vi "OwnMergeDiagram_75a8ff880a4e45db8adbb9b45fd37ec5.vi"() -> ()   [LabVIEW 2024]
doc: "该范例演示VI脚本的“移动选定对象”方法，以编程方式在编辑环境下触发鼠标拖动。这是移动多个对象的有效方法。\n\n将'Duplicate?'参数的值设置为TRUE，移动操作就可以成为复制操作。"
uses:
  <vilib>/Utility/miscctls.llb/LVDeltaXY32Cluster.ctl
panel:
  out "selected_source_objects":refnum<vi>[](array[refnum])
  out "error out":errorcluster caption="错误输出"
  in  "delta":T1 caption="X/Y Delta"
  in  "target_path":path
  in  "source_path":path
  # "概述：演示VI脚本中的移动选定对象方法，将当前选定区域移动至其他位置\n操作步骤：\n1.打开Test - Selection List Target.vi的程序框图。\n2.选择一个或多个对象。\n3.运行本VI。选中的对象将在程序框图上向上移动25个像素。"
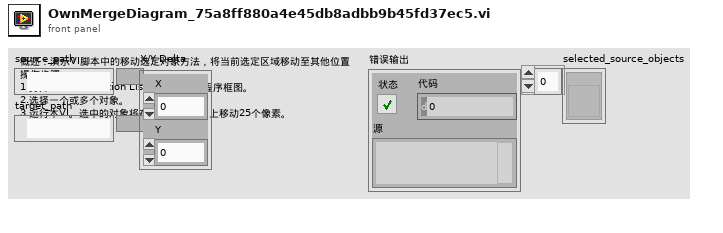
[diagram p1: front panel]
types:
  T1 = typedef "LVDeltaXY32Cluster.ctl" = cluster{"X":i32, "Y":i32}
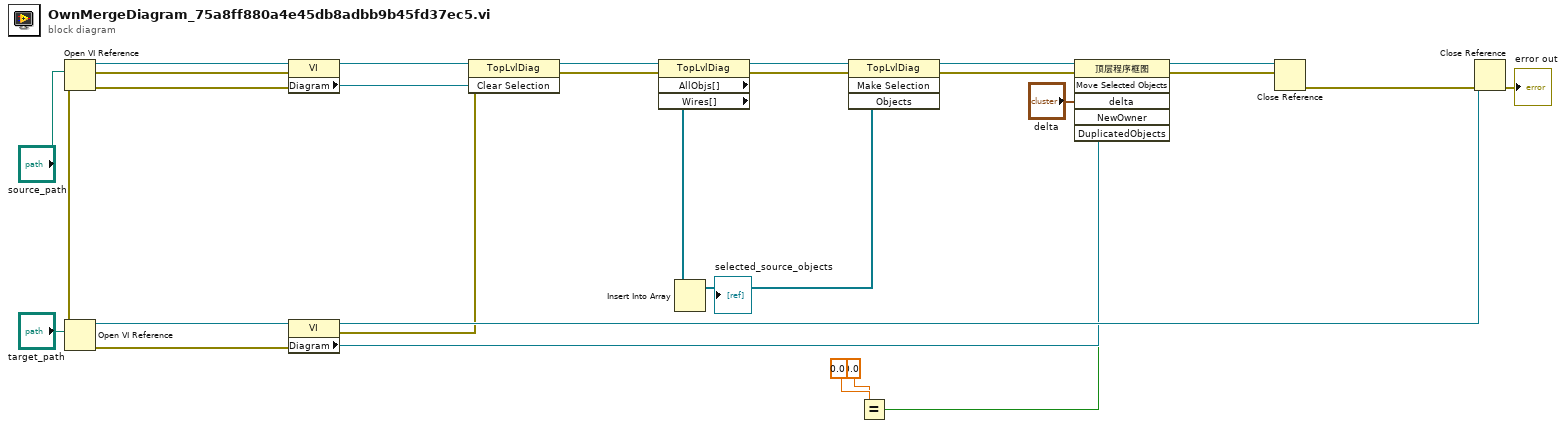
[diagram p0: block diagram]
diagram:
  n1 = Open VI Reference(vi path="source_path") -> (vi reference=w25:refnum<vi>, error out=w24:errorcluster)  [unwired: 5 in]
  n2 = property class="VI"(reference=w25, error in=w24) -> (error out=w22:errorcluster, "Diagram"=w19:refnum<vi>)  [unwired: 1 out]
  n3 = Open VI Reference(vi path="target_path", error in (no error)=w22) -> (vi reference=w21:refnum<vi>, error out=w20:errorcluster)  [unwired: 4 in]
  n4 = property class="VI"(reference=w21, error in=w20) -> (error out=w18:errorcluster, "Diagram"=w8:refnum<vi>)  [unwired: 1 out]
  n5 = invoke class="TopLvlDiag" method="Clear Selection"(reference=w19, error in=w18) -> (reference out=w17:refnum<vi>, error out=w16:errorcluster)  [unwired: 1 in, 1 out]
  n6 = property class="TopLvlDiag"(reference=w17, error in=w16) -> (reference out=w13:refnum<vi>, error out=w11:errorcluster, "AllObjs[]"=w15:refnum<vi>[], "Wires[]"=w14:refnum<vi>[])
  n7 = Insert Into Array(array=w15, new element=w14) -> (w12:refnum<vi>[])  [unwired: 1 in]
  "selected_source_objects" <- w12
  n8 = invoke class="TopLvlDiag" method="Make Selection"(reference=w13, error in=w11, "Objects"=w12) -> (reference out=w10:refnum<vi>, error out=w9:errorcluster)  [unwired: 1 in, 2 out]
  n9 = Equal?(x=0.0, y=0.0) -> (x = y?=w4:bool)
  n10 = invoke class="顶层程序框图" method="Move Selected Objects"(reference=w10, error in=w9, "delta"="delta", "NewOwner"=w8, "DuplicatedObjects"=w4) -> (error out=w3:errorcluster)  [unwired: 1 in, 5 out]
  n11 = Close Reference(reference=w25, error in (no error)=w3) -> (error out=w2:errorcluster)
  n12 = Close Reference(reference=w21, error in (no error)=w2) -> (error out=→"error out":errorcluster)
